vi "SelectPatternDialog.vi"(0 "GraphIn":refnum<class "Graph.lvclass">, 1 "SelectedNodes":refnum<class "AbstractNode.lvclass">[](array[class]), 5 "error in":errorcluster) -> (14 "GraphOut":refnum<class "Graph.lvclass">, 15 "Cancelled":bool, 16 "NodesOut":T3[](array[typedef]), 17 "LinksOut":T1[](array[typedef]), 18 "NodeIndexies":i32[](array[numeric]), 19 "error out":errorcluster)   [LabVIEW 2020]
uses:
  <resource>/Framework/Providers/Open_GDS/UML/Graph_class/Graph.lvclass
  <resource>/Framework/Providers/Open_GDS/UML/AbstractNode_class/AbstractNode.lvclass
  <resource>/Framework/Providers/Open_GDS/UML/DesignPattern/SubVIs/DesignPatterns_Node.ctl
  <resource>/Framework/Providers/Open_GDS/UML/DesignPattern/SubVIs/DesignPatterns_NodeType.ctl
  <resource>/Framework/Providers/Open_GDS/UML/DesignPattern/SubVIs/DesignPatterns_Link.ctl
  <resource>/Framework/Providers/Open_GDS/UML/DesignPattern/SubVIs/DesignPatterns_LinkType.ctl
  <resource>/Framework/Providers/Open_GDS/UML/Graphics_class/Graphics.lvclass
  <resource>/Framework/Providers/Open_GDS/UML/Grid_class/Grid.lvclass
  <resource>/Framework/Providers/Open_GDS/UML/ClassDiagramGraph_class/ClassDiagramGraph.lvclass
  C:/Program Files (x86)/National Instruments/LabVIEW 2020/resource/Framework/Providers/Open_GDS/UML/Graph_class/Graph.lvclass
  <resource>/Framework/Providers/Open_GDS/UML/DesignPattern/SubVIs/DesignPatterns_Pattern.ctl
  <resource>/Framework/Providers/Open_GDS/UML/Graphics_class/LvFontType.ctl
  <resource>/Framework/Providers/Open_GDS/UML/Graphics_class/FontType.ctl
  <resource>/Framework/Providers/Open_GDS/UML/ClassNode_class/ClassNode.lvclass
  <resource>/Framework/Providers/Open_GDS/UML/DesignPattern/SubVIs/DesignPatterns_ClassNodeData.ctl
  <resource>/Framework/Providers/Open_GDS/UML/DesignPattern/SubVIs/DesignPatterns_Attribute.ctl
  <resource>/Framework/Providers/Open_GDS/UML/DesignPattern/SubVIs/DesignPatterns_Method.ctl
  <vilib>/Platform/browser.llb/Open URL in Default Browser (string).vi
panel:
  in  "OpenPatternFile":bool
  in  "Refresh":bool
  in  "Ring 10":u16(ring) items=["<Select>"]
  in  "Ring 9":u16(ring) items=["<Select>"]
  in  "Ring 8":u16(ring) items=["<Select>"]
  in  "Ring 7":u16(ring) items=["<Select>"]
  in  "Help":bool
  in  "Cancel":bool
  in  "OK":bool
  out "Nodes":cluster{"Name":string, "Desc":string}[](array[cluster])
  out "Pattern description":string
  out "NewVal":string
  in  "Design Patterns":string(tree)
  in  "InterfaceNames":string[](array[string])
  in  "PackageNames":string[](array[string])
  out "ClassNames":string[](array[string])
  in  "Ring 6":u16(ring) items=["<Select>"]
  in  "Ring 5":u16(ring) items=["<Select>"]
  in  "Ring 4":u16(ring) items=["<Select>"]
  in  "Ring 3":u16(ring) items=["<Select>"]
  in  "Ring 2":u16(ring) items=["<Select>"]
  in  "Ring 1":u16(ring) items=["<Select>"]
  out "Picture":picture
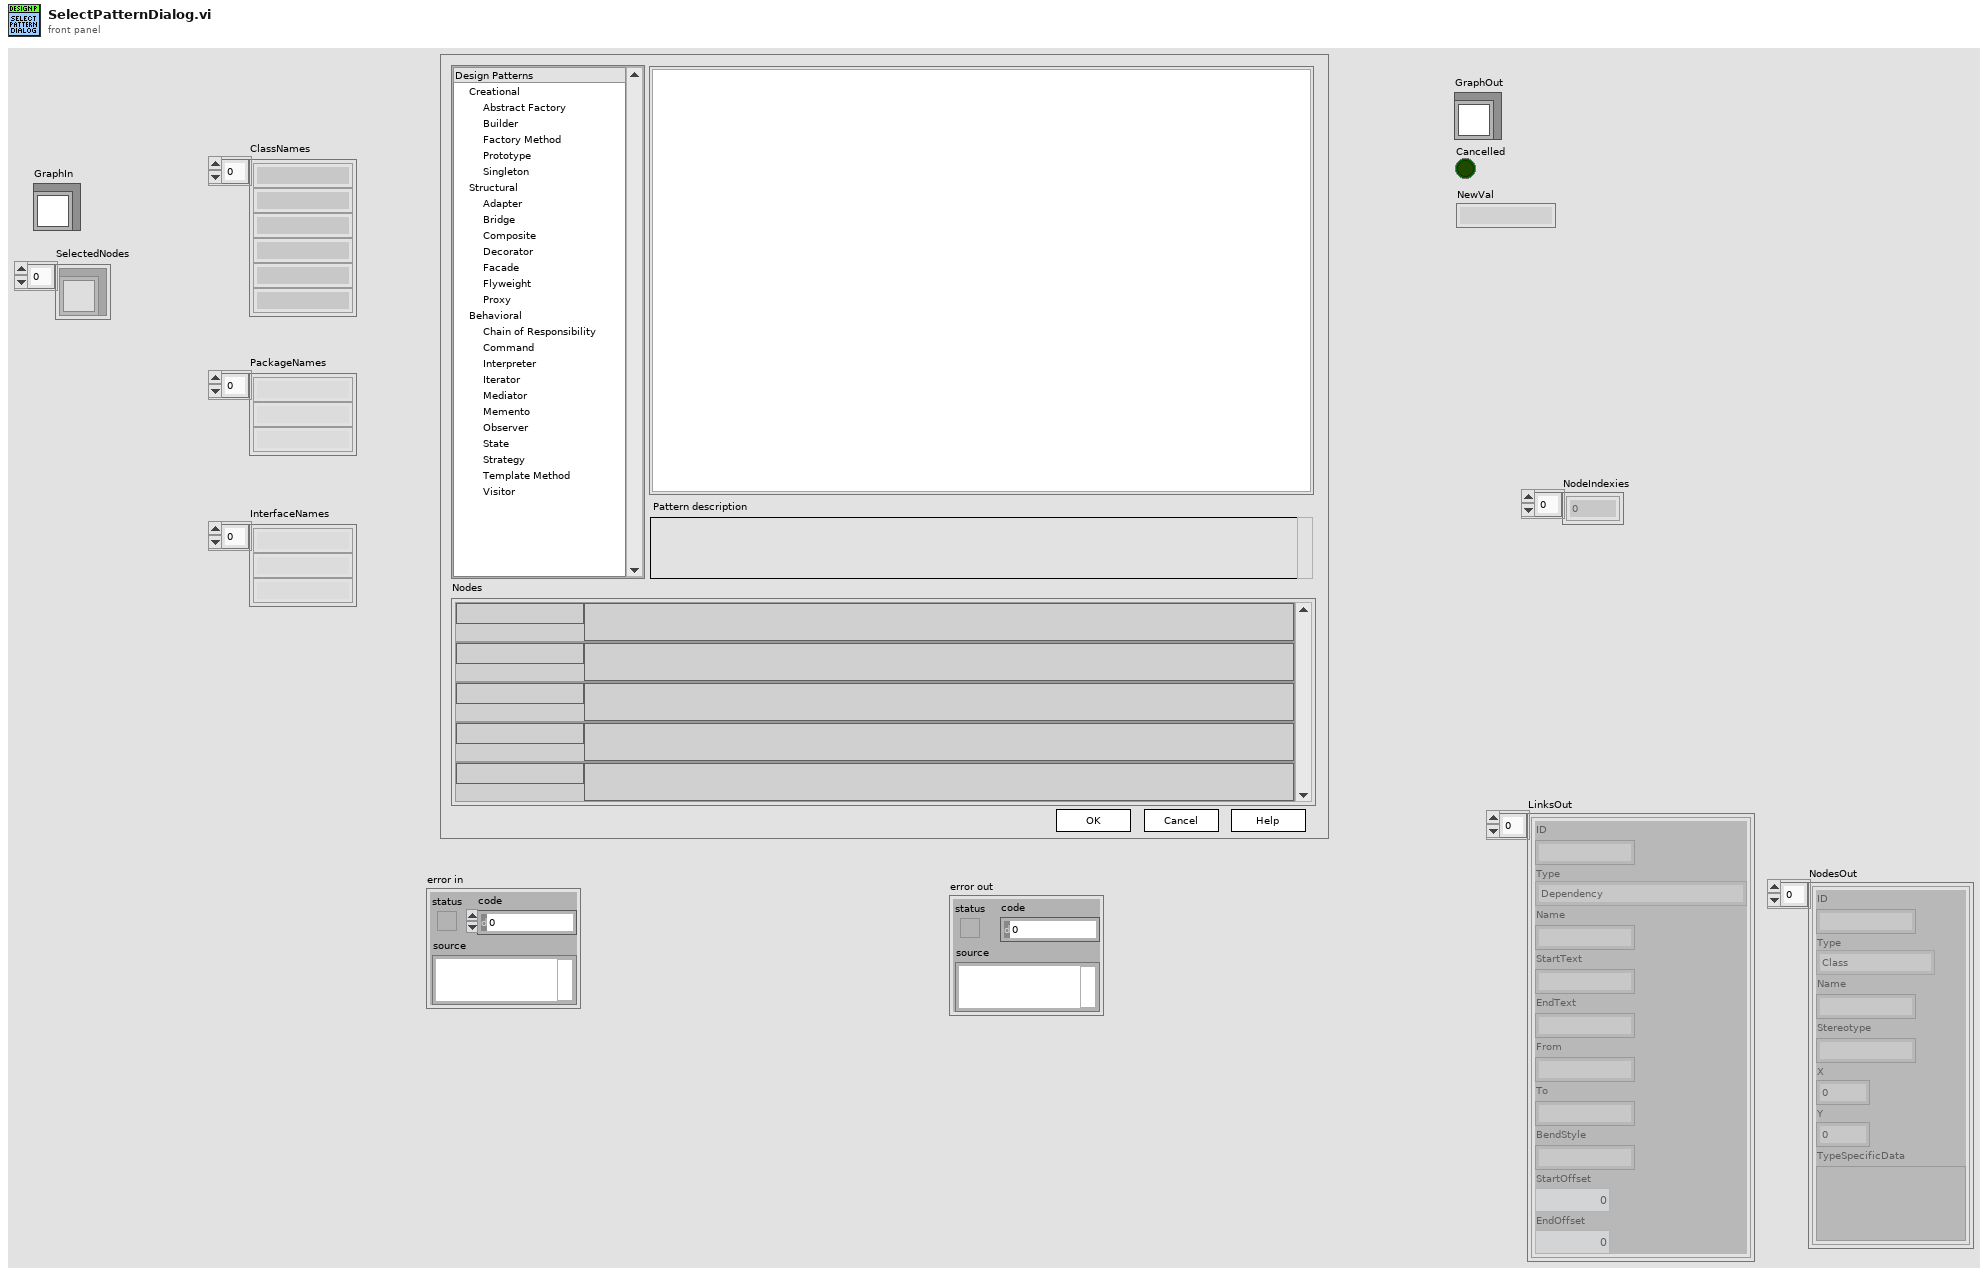
[diagram p1: front panel]
types:
  T1 = typedef "DesignPatterns_Link.ctl" = cluster{"ID":string, "Type":T2, "Name":string, "StartText":string, "EndText":string, "From":string, "To":string, "BendStyle":string, "StartOffset":i32, "EndOffset":i32}
  T2 = typedef "DesignPatterns_LinkType.ctl" = enum16{"Dependency", "Inheritance", "Interface", "Association", "Aggregation", "CompositeAggregation"}
  T3 = typedef "DesignPatterns_Node.ctl" = cluster{"ID":string, "Type":T4, "Name":string, "Stereotype":string, "X":i32, "Y":i32, "TypeSpecificData":variant}
  T4 = typedef "DesignPatterns_NodeType.ctl" = enum16{"Class", "Interface", "Note", "Package"}
  T5 = typedef "DesignPatterns_Pattern.ctl" = cluster{"Version":string, "ID":string, "Name":string, "Category":string, "Help":string, "Desc":string}
  T6 = cluster{"Cancelled":bool, "Event":refnum<event-registration>, "CtrlRefs":refnum<vi>[], "PIDs":string[], "Graphics":refnum<class "Graphics.lvclass">, "Grid":refnum<class "Grid.lvclass">, "Diagram":refnum<class "ClassDiagramGraph.lvclass">, "ClassNodes":T3[], "ClassSelected":bool[], "NodeIndexies":i32[], "Patterns":cluster{"PatternFile":path, "Pattern":T5, "Nodes":T3[], "Links":T1[], "stripped path":path, "HelpExist":bool}[], "Interface?":bool[]}
  T7 = typedef "Graphics.lvclass/FontType.ctl" = cluster{"Font Name:":string, "Size":i16, "Strikeout?":bool, "Italic?":bool, "Underline?":bool, "Outline?":bool, "Shadow?":bool, "Bold?":bool}
  T8 = typedef "Graphics.lvclass/LvFontType.ctl" = enum16{"User-specified Font", "Application Font", "System Font", "Dialog Font"}
  T9 = cluster{path, "Pattern":T5, "Nodes":T3[], "Links":T1[], "stripped path":path, "file or folder exists?":bool}[]
  T10 = typedef "DesignPatterns_ClassNodeData.ctl" = cluster{"Description":string, "Attributes":T11[], "Methods":T12[]}
  T11 = typedef "DesignPatterns_Attribute.ctl" = cluster{"ID":string, "Name":string}
  T12 = typedef "DesignPatterns_Method.ctl" = cluster{"ID":string, "Name":string}
  T13 = typedef "Rectangle Rectangle2D.ctl" = cluster{"x":dbl, "y":dbl, "width":dbl, "height":dbl}
  T14 = cluster{path, "Pattern":T5, "Nodes":T3[], "Links":T1[], "stripped path":path, "file or folder exists?":bool}
  T15 = cluster{"PatternFile":path, "Pattern":T5, "Nodes":T3[], "Links":T1[], "stripped path":path, "HelpExist":bool}[]
  T16 = cluster{"PatternFile":path, "Pattern":T5, "Nodes":T3[], "Links":T1[], "stripped path":path, "HelpExist":bool}
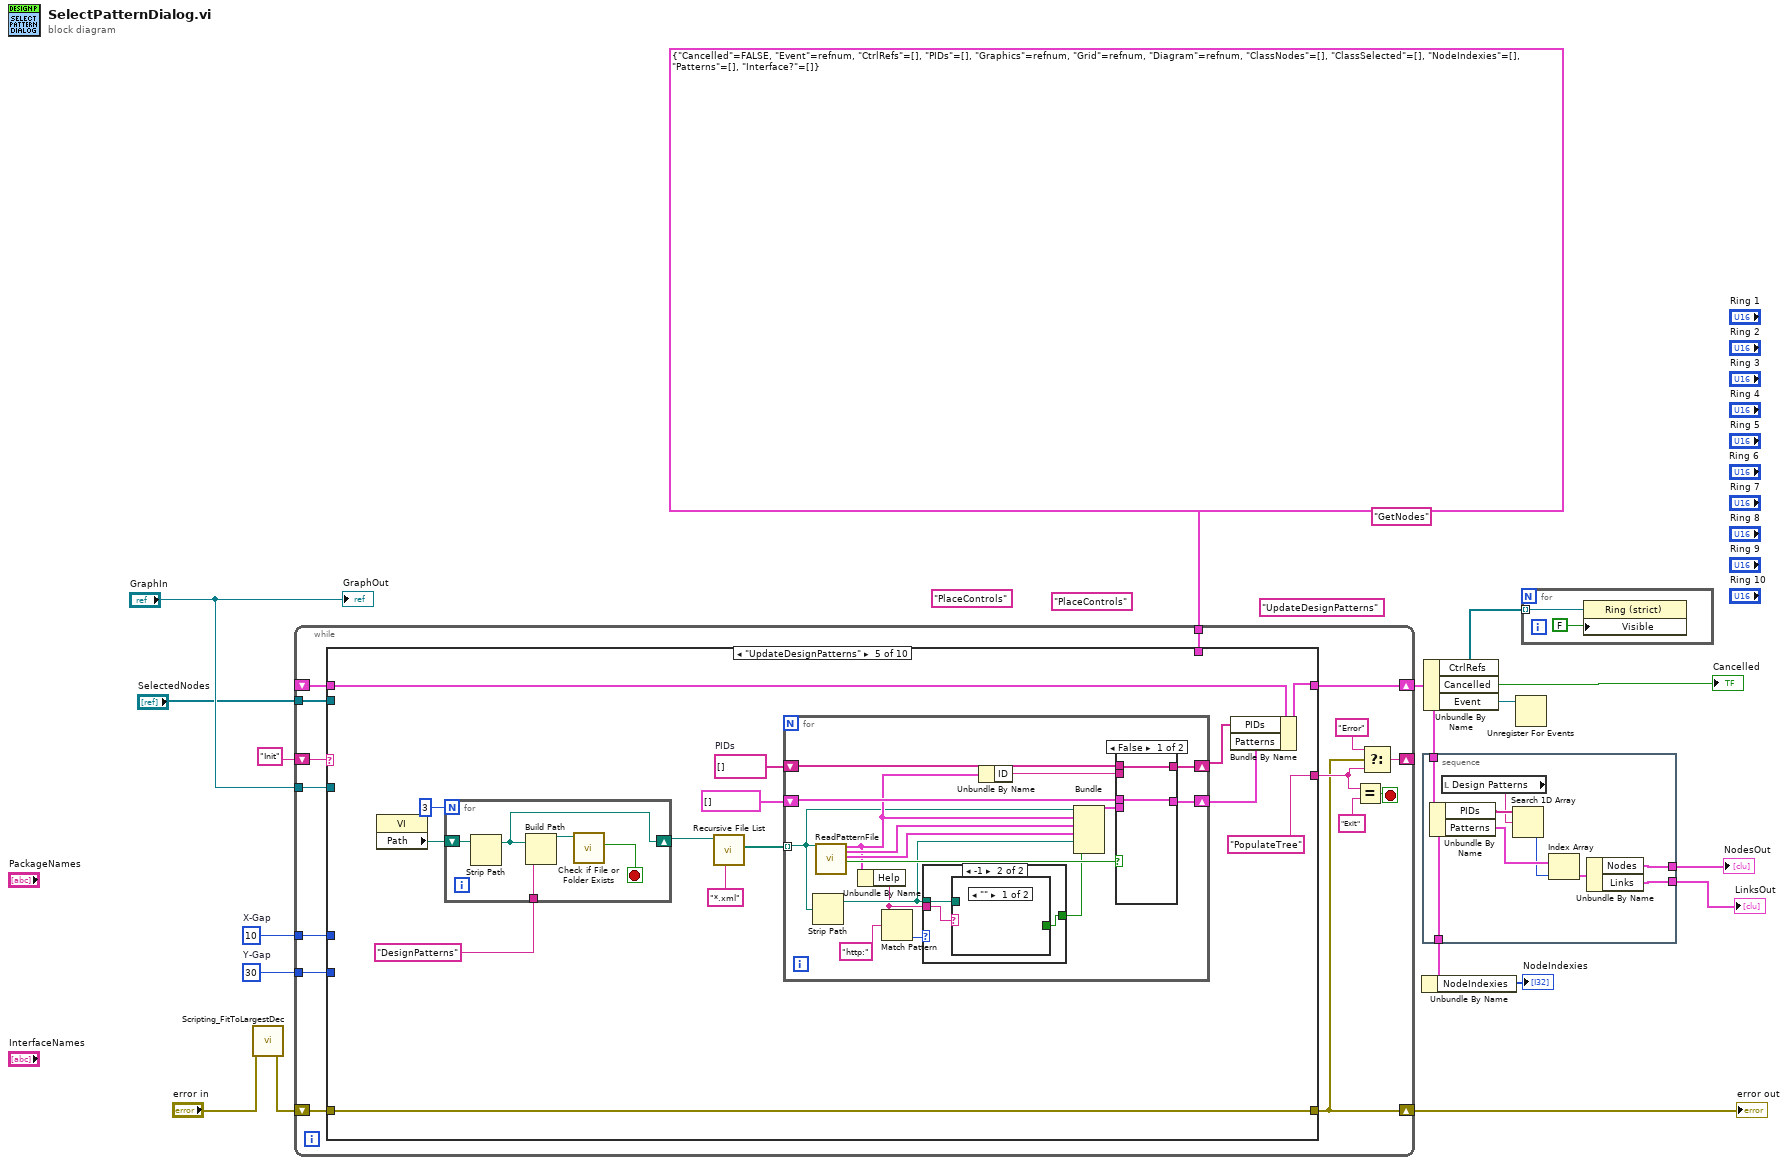
[diagram p0: block diagram]
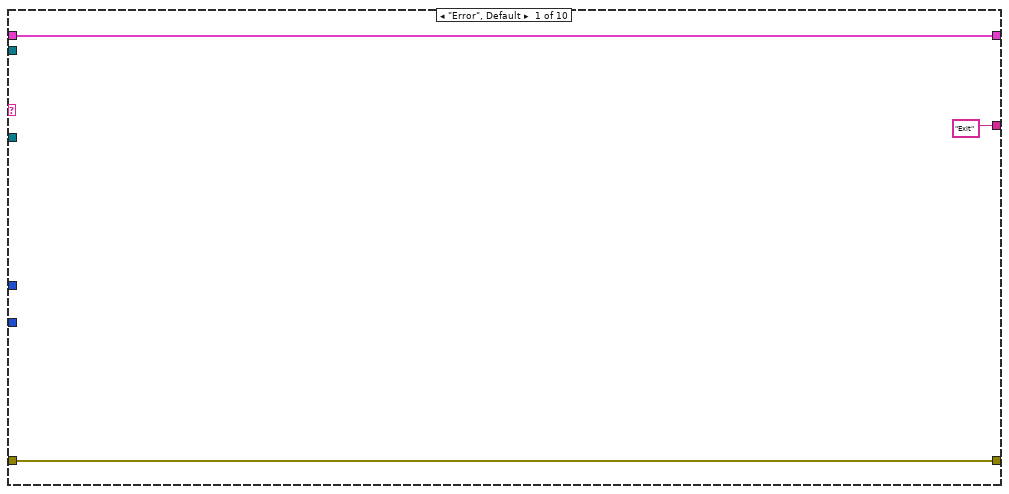
[diagram p2: hidden frame]
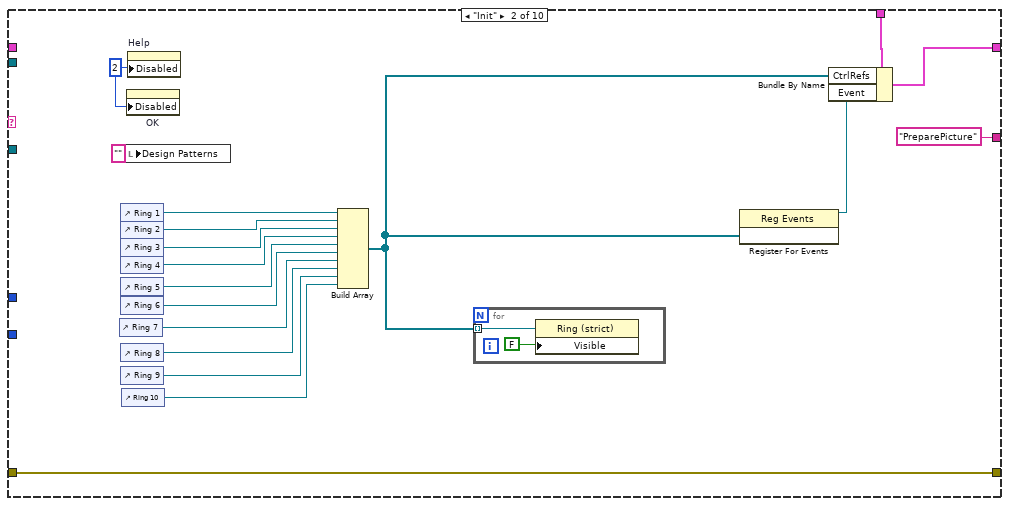
[diagram p3: hidden frame]
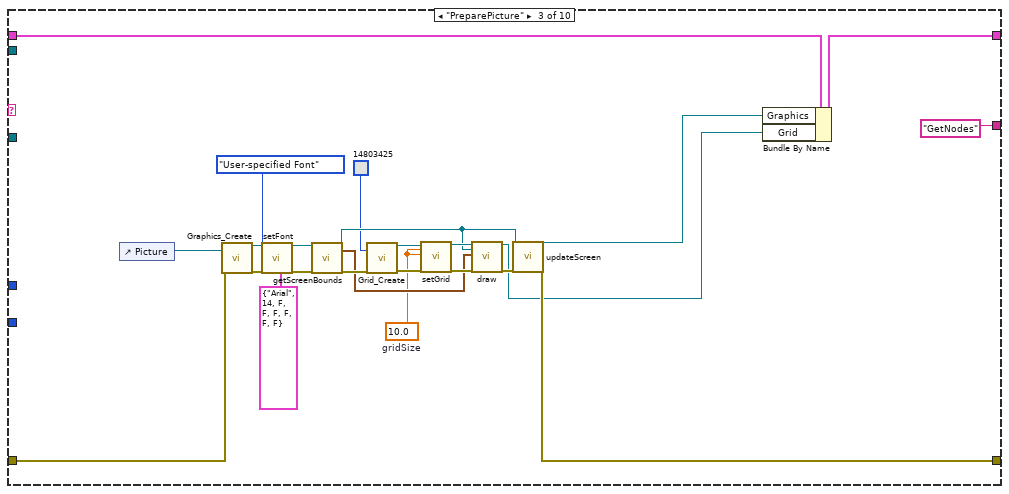
[diagram p4: hidden frame]
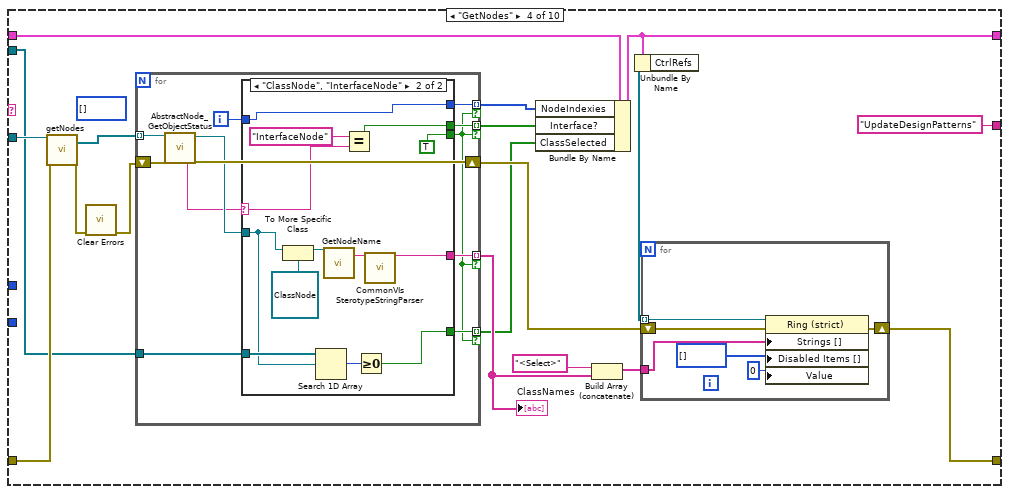
[diagram p5: hidden frame]
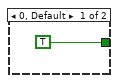
[diagram p7: hidden frame]
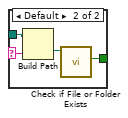
[diagram p8: hidden frame]
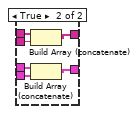
[diagram p9: hidden frame]
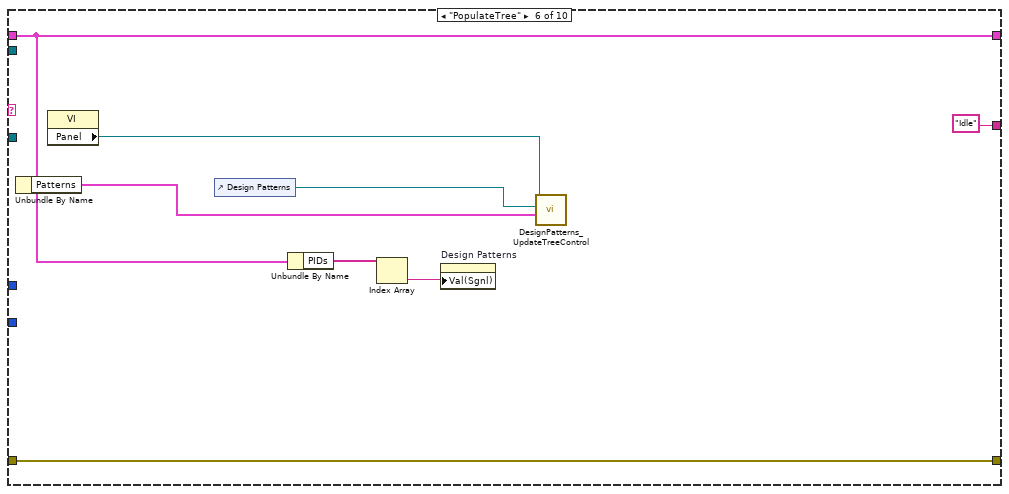
[diagram p10: hidden frame]
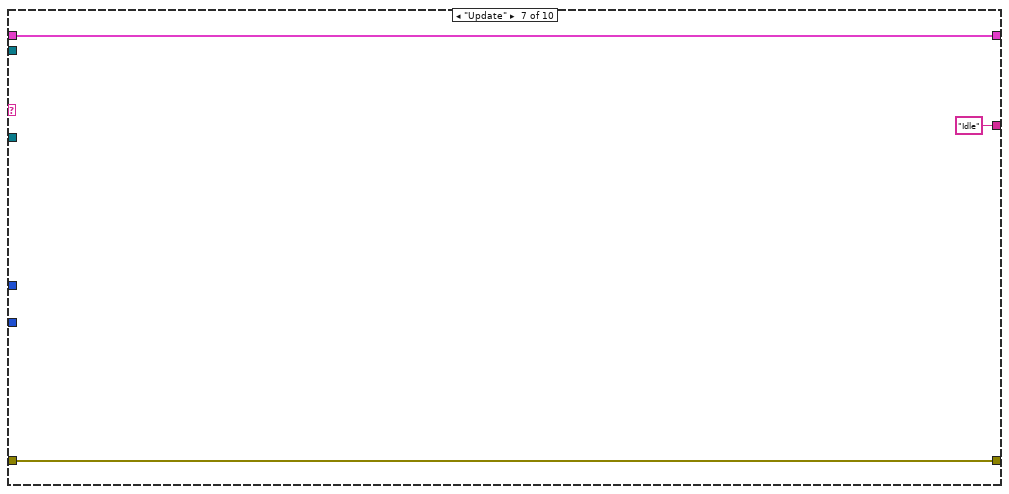
[diagram p11: hidden frame]
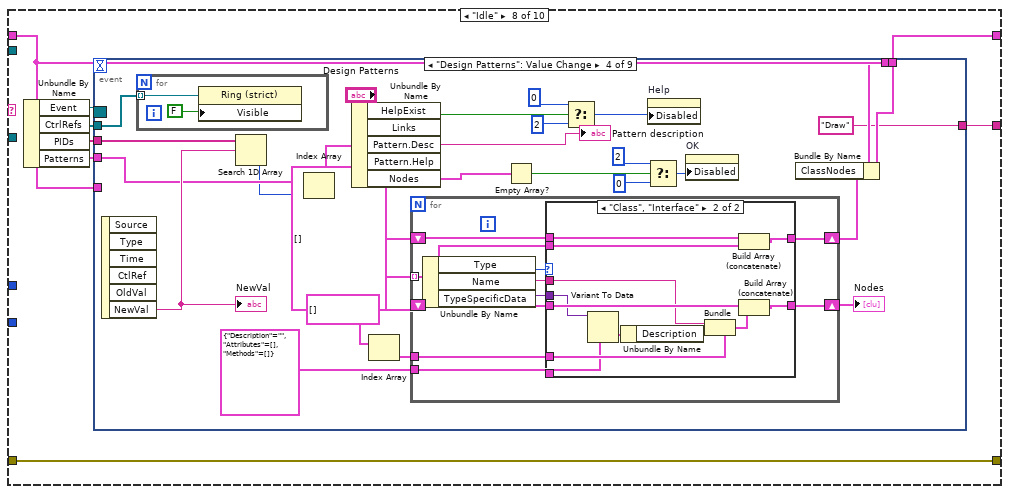
[diagram p12: hidden frame]
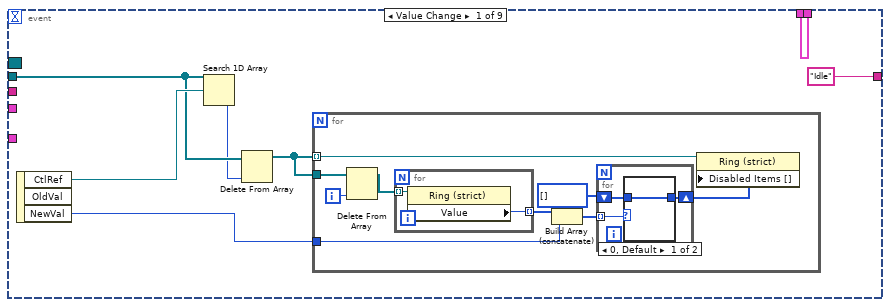
[diagram p13: hidden frame]
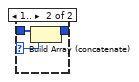
[diagram p14: hidden frame]
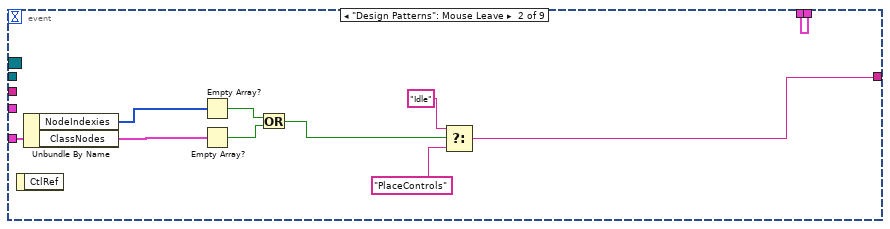
[diagram p15: hidden frame]
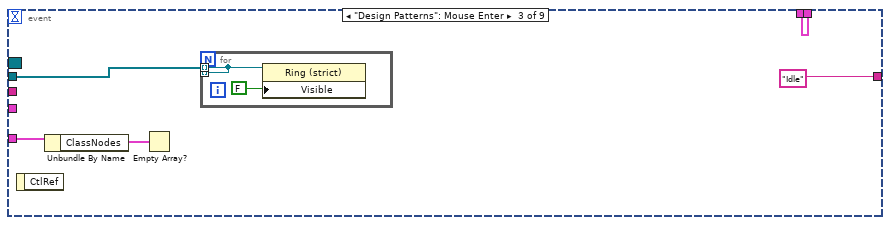
[diagram p16: hidden frame]
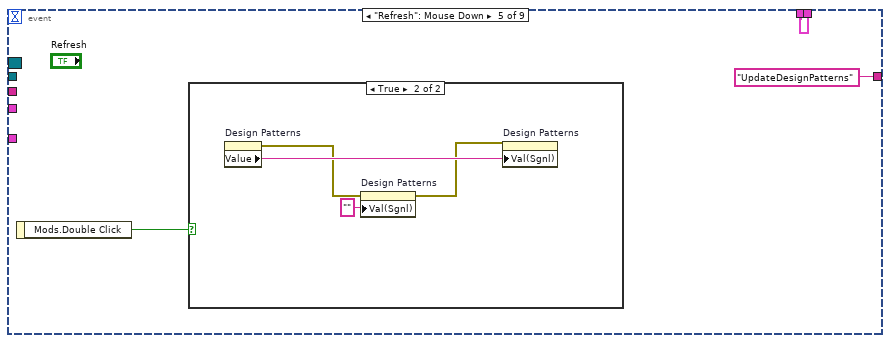
[diagram p18: hidden frame]
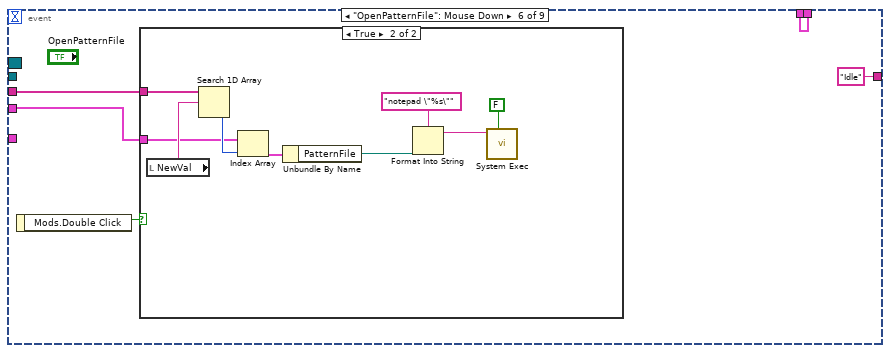
[diagram p20: hidden frame]
diagram:
  (unwired) "PlaceControls"
  w8 = 30  # Y-Gap
  w9 = 10  # X-Gap
  (unwired) "GetNodes"
  (unwired) "UpdateDesignPatterns"
  (unwired) "PlaceControls"
  n1 = call <resource>:"Scripting_FitToLargestDec.vi"("error in (no error)"="error in") -> ("error out"=w10:errorcluster)  [unwired: 5 in, 1 out]
  n2 = while {
    shift-right: [w25] -> w16
    shift-left: w10 -> [w32]
    shift-right: [w30] -> _
    shift-left: "Init" -> [w31]
    shift-right: [w24] -> w6
    shift-left: _ -> [w23]
    tunnel: T6 {"Cancelled"=FALSE, "Event"=refnum, "CtrlRefs"=[], "PIDs"=[], "Graphics"=refnum, "Grid"=refnum, "Diagram"=refnum, "ClassNodes"=[], "ClassSelected"=[], "NodeIndexies"=[], "Patterns"=[], "Interface?"=[]} -> [w22]
    tunnel: "GraphIn" -> [w21]
    tunnel: w9 -> [w20]
    tunnel: w8 -> [w19]
    tunnel: "SelectedNodes" -> [w18]
    stop <- w29 stop-if-true
    n3 = case shown="\"UpdateDesignPatterns\"" w31 {
      tunnel: w32 -> [w35 w52 w63 w91 w132 w185 w188 w196 w365 w405]
      tunnel: [w35 w52 w62 w90 w132 w185 w188 w196 w367 w401] -> w25
      tunnel: ["Exit" "PreparePicture" "GetNodes" "UpdateDesignPatterns" "PopulateTree" "Idle" "Idle" w197 "Idle" "Idle"] -> w26
      tunnel: [w33 w51 w56 w86 w134 w182 w189 w198 w387 w399] -> w24
      tunnel: w23 -> [w33 _ w57 w87 w136 w182 w189 w191 w387 w399]
      tunnel: w22 -> [_ w43 _ _ _ _ _ _ _ _]
      tunnel: w21 -> [_ _ _ w93 _ _ _ _ _ _]
      tunnel: w20 -> [_ _ _ _ _ _ _ _ w360 w412]
      tunnel: w19 -> [_ _ _ _ _ _ _ _ w359 w411]
      tunnel: w18 -> [_ _ _ w88 _ _ _ _ _ w404]
      frame "Error", Default {
      }
      frame "Init" {
        w42 = u8 2 ("Disabled")
        n4 = control-ref of="Ring 7"() -> (w39:refnum<vi>)
        n5 = control-ref of="Ring 1"() -> (w45:refnum<vi>)
        n6 = control-ref of="Ring 2"() -> (w46:refnum<vi>)
        n7 = control-ref of="Ring 3"() -> (w47:refnum<vi>)
        n8 = control-ref of="Ring 4"() -> (w48:refnum<vi>)
        n9 = control-ref of="Ring 5"() -> (w49:refnum<vi>)
        n10 = control-ref of="Ring 6"() -> (w50:refnum<vi>)
        n11 = control-ref of="Ring 8"() -> (w38:refnum<vi>)
        n12 = control-ref of="Ring 9"() -> (w37:refnum<vi>)
        n13 = control-ref of="Ring 10"() -> (w36:refnum<vi>)
        n14 = local write "Design Patterns"("" ("Design Patterns")) -> ()
        n15 = property on="OK" class="Bool"("Disabled"=w42) -> ()  [unwired: 2 in, 2 out]
        n16 = property on="Help" class="Bool"("Disabled"=w42) -> ()  [unwired: 2 in, 2 out]
        n17 = Build Array(w45, w46, w47, w48, w49, w50, w39, w38, w37, w36) -> (w40:refnum<vi>[])
        n18 = for {
          tunnel: w40 -> [w55] mode=indexing
          n19 = property class="Ring (strict)"(reference=w55, "Visible"=FALSE) -> ()  [unwired: 1 in, 2 out]
        }
        n20 = register-events(w40) -> (reference out=w44:refnum<event-registration>)  [unwired: 2 in, 1 out]
        n21 = Bundle By Name(cluster=w43, "CtrlRefs"=w40, "Event"=w44) -> (w51:T6)
      }
      frame "PreparePicture" {
        w64 = 10.0  # gridSize
        n22 = control-ref of="Picture"() -> (w60:refnum<vi>)
        n23 = call <resource>:"Graphics_Create.vi"("screenRef"=w60, "error in (no error)"=w63) -> ("reference out"=w73:refnum<class "Graphics.lvclass">, "error out"=w72:errorcluster)  [unwired: 1 in, 15 out]
        n24 = call <resource>:"setFont.vi"("reference"=w73, "fontType"=LvFontType."User-specified Font", "font"=T7 {"Font Name:"="Arial", "Size"=14, "Strikeout?"=FALSE, "Italic?"=FALSE, "Underline?"=FALSE, "Outline?"=FALSE, "Shadow?"=FALSE, "Bold?"=FALSE}, "error in (no error)"=w72) -> ("reference out"=w71:refnum<class "Graphics.lvclass">, "error out"=w70:errorcluster)  [unwired: 14 out]
        n25 = call <resource>:"getScreenBounds.vi"("reference"=w71, "error in (no error)"=w70) -> ("reference out"=w74:refnum<class "Graphics.lvclass">, "bounds"=w67:T13, "error out"=w79:errorcluster)  [unwired: 15 out]
        n26 = call <resource>:"Grid_Create.vi"("gridColor"=u32 14803425, "error in (no error)"=w79) -> ("reference out"=w76:refnum<class "Grid.lvclass">, "error out"=w77:errorcluster)  [unwired: 1 in, 15 out]
        n27 = call <resource>:"setGrid.vi"("reference"=w76, "gridX"=w64, "gridY"=w64, "error in (no error)"=w77) -> ("reference out"=w75:refnum<class "Grid.lvclass">, "error out"=w78:errorcluster)  [unwired: 14 out]
        n28 = call-dynamic "draw.vi"("reference"=w75, "graphics"=w74, "bounds"=w67, "error in (no error)"=w78) -> ("reference out"=w58:refnum<class "Grid.lvclass">, "error out"=w66:errorcluster)  [unwired: 14 in]
        n29 = call <resource>:"updateScreen.vi"("reference"=w74, "error in (no error)"=w66) -> ("reference out"=w59:refnum<class "Graphics.lvclass">, "error out"=w62:errorcluster)  [unwired: 16 out]
        n30 = Bundle By Name(cluster=w57, "Graphics"=w59, "Grid"=w58) -> (w56:T6)
      }
      frame "GetNodes" {
        (unwired) i32[] []
        n31 = call-dynamic "getNodes.vi"("reference"=w93, "error in (no error)"=w91) -> ("nodes"=w92:refnum<class "AbstractNode.lvclass">[], "error out"=w81:errorcluster)  [unwired: 15 in, 1 out]
        n32 = call <vilib>:"Clear Errors.vi"("error in (no error)"=w81) -> ("error out"=w80:errorcluster)  [unwired: 5 in, 1 out]
        n33 = for {
          shift-right: [w107] -> w89
          shift-left: w80 -> [w109]
          tunnel: w92 -> [w108] mode=indexing
          tunnel: w88 -> [w105]
          tunnel: [w102] -> w85 mode=indexing if=w98
          tunnel: [w101] -> w84 mode=indexing if=w98
          tunnel: [w100] -> w83 mode=indexing if=w98
          tunnel: [w99] -> w82 mode=indexing if=w98
          i -> [w104]
          n34 = call <resource>:"AbstractNode_GetObjectStatus.vi"("reference in"=w108, "error in (no error)"=w109) -> ("Class name"=w103:string, "reference out"=w106:refnum<class "AbstractNode.lvclass">, "error out"=w107:errorcluster)  [unwired: 15 out]
          n35 = case shown="\"ClassNode\", \"InterfaceNode\"" w103 {
            selector: w103 -> [_ w116]
            tunnel: w106 -> [_ w118]
            tunnel: w105 -> [_ w119]
            tunnel: [_ w112] -> w101
            tunnel: w104 -> [_ w112]
            tunnel: [_ w114] -> w102
            tunnel: [_ TRUE] -> w98
            tunnel: [_ w111] -> w100
            tunnel: [_ w110] -> w99
            frame Default {
            }
            frame "ClassNode", "InterfaceNode" {
              n36 = To More Specific Class(target class=refnum<class "ClassNode.lvclass"> refnum ("reference"), reference=w118) -> (specific class reference=w121:refnum<class "ClassNode.lvclass">)  [unwired: 1 in, 1 out]
              n37 = Search 1D Array(1D array=w119, element=w118) -> (index of element=w117:i32)  [unwired: 1 in]
              n38 = call-dynamic "GetNodeName.vi"("reference in"=w121) -> ("String"=w120:string)  [unwired: 16 in, 2 out]
              n39 = Equal?(x="InterfaceNode", y=w116) -> (x = y?=w114:bool)
              n40 = Greater Or Equal To 0?(x=w117) -> (x >= 0?=w110:bool)
              n41 = call <resource>:"CommonVIs SterotypeStringParser.vi"("SterotypeStringIn"=w120) -> ("Name"=w111:string)  [unwired: 18 out]
            }
          }
        }
        "ClassNames" <- w83
        n42 = Bundle By Name(cluster=w87, "NodeIndexies"=w84, "Interface?"=w85, "ClassSelected"=w82) -> (w86:T6)
        n43 = Build Array (concatenate)("<Select>", w83) -> (w96:string[])
        n44 = Unbundle By Name(w86) -> ("CtrlRefs"=w95:refnum<vi>[])
        n45 = for {
          tunnel: w95 -> [w128] mode=indexing
          tunnel: w96 -> [w127]
          shift-right: [w123] -> w90
          shift-left: w89 -> [w124]
          n46 = property class="Ring (strict)"(reference=w128, error in=w124, "Strings []"=w127, "Disabled Items []"=i32[] [], "Value"=u16 0) -> (error out=w123:errorcluster)  [unwired: 1 out]
        }
      }
      frame "UpdateDesignPatterns" {
        w131 = string[] []  # PIDs
        n47 = property class="VI"() -> ("Path"=w140:path)  [unwired: 2 in, 2 out]
        n48 = for {
          N: 3 -> [_]
          tunnel: "DesignPatterns" ("name or relative path") -> [w179]
          shift-right: [w175] -> w139
          shift-left: w140 -> [w176]
          stop <- w177 stop-if-true
          n49 = Strip Path(path=w176) -> (stripped path=w175:path)  [unwired: 1 out]
          n50 = Build Path(base path=w175, name or relative path=w179) -> (appended path=w178:path)
          n51 = call <vilib>:"Check if File or Folder Exists.vi"("path"=w178) -> ("file or folder exists?"=w177:bool)  [unwired: 1 in, 9 out]
        }
        n52 = call <vilib>:"Recursive File List.vi"("pattern"="*.xml", "Folder Path"=w139) -> ("All Files in Dir"=w137:path[])  [unwired: 2 in, 7 out]
        n53 = for {
          tunnel: w137 -> [w143] mode=indexing
          shift-right: [w154] -> w135
          shift-left: T9 [] -> [w156]
          shift-right: [w151] -> w130
          shift-left: w131 -> [w150]
          n54 = Strip Path(path=w143) -> (stripped path=w145:path)  [unwired: 1 out]
          n55 = call <resource>:"ReadPatternFile.vi"("PatternsXMLFileIn"=w143) -> ("Pattern"=w149:T5, "Nodes"=w158:T3[], "Links"=w157:T1[], "Valid"=w153:bool)  [unwired: 2 in, 13 out]
          n56 = Unbundle By Name(w149) -> ("Help"=w144:string)
          n57 = Match Pattern(string=w144, regular expression="http:") -> (offset past match=w147:i32)  [unwired: 4 out]
          n58 = case shown="-1" w147 {
            tunnel: [TRUE w160] -> w146
            tunnel: w145 -> [_ w162]
            tunnel: w144 -> [_ w161]
            frame 0, Default {
            }
            frame -1 {
              n59 = case shown="\"\"" w161 {
                selector: w161 -> [_ w164]
                tunnel: w162 -> [_ w165]
                tunnel: [_ w163] -> w160
                frame "" {
                }
                frame Default {
                  n60 = Build Path(base path=w165, name or relative path=w164) -> (appended path=w166:path)
                  n61 = call <vilib>:"Check if File or Folder Exists.vi"("path"=w166) -> ("file or folder exists?"=w163:bool)  [unwired: 1 in, 9 out]
                }
              }
            }
          }
          n62 = Unbundle By Name(w149) -> ("ID"=w152:string)
          n63 = Bundle(w143, "Pattern"=w149, "Nodes"=w158, "Links"=w157, "stripped path"=w145, "file or folder exists?"=w146) -> (w155:T14)  [unwired: 1 out]
          n64 = case shown="False" w153 {
            tunnel: w156 -> [w168 w174]
            tunnel: w155 -> [_ w173]
            tunnel: [w168 w172] -> w154
            tunnel: w152 -> [_ w171]
            tunnel: [w167 w170] -> w151
            tunnel: w150 -> [w167 w169]
            frame False {
            }
            frame True {
              n65 = Build Array (concatenate)(w169, w171) -> (w170:string[])
              n66 = Build Array (concatenate)(w174, w173) -> (w172:T9)
            }
          }
        }
        n67 = Bundle By Name(cluster=w136, "PIDs"=w130, "Patterns"=w135) -> (w134:T6)
      }
      frame "PopulateTree" {
        n68 = Unbundle By Name(w182) -> ("Patterns"=w184:T15)
        n69 = property class="VI"() -> ("Panel"=w187:refnum<vi>)  [unwired: 2 in, 2 out]
        n70 = control-ref of="Design Patterns"() -> (w183:refnum<vi>)
        n71 = Unbundle By Name(w182) -> ("PIDs"=w181:string[])
        n72 = Index Array(array=w181) -> (element=w180:string)  [unwired: 1 in]
        n73 = property on="Design Patterns" class="Tree (strict)"("Val(Sgnl)"=w180) -> ()  [unwired: 2 in, 2 out]
        n74 = call <resource>:"DesignPatterns_UpdateTreeControl.vi"("Patterns"=w184, "Tree Refnum"=w183, "Panel"=w187) -> ()  [unwired: 9 out]
      }
      frame "Update" {
      }
      frame "Idle" {
        n75 = Unbundle By Name(w191) -> ("Event"=w195:refnum<event-registration>, "CtrlRefs"=w194:refnum<vi>[], "PIDs"=w193:string[], "Patterns"=w192:T15)
        n76 = event shown="[3] \"Design Patterns\": Value Change" {
          selector: w195 -> [_ _ _ _ _ _ _ _ _]
          dyn-events: _ -> [_ _ _ _ _ _ _ _ _]
          timeout: _ -> [_ _ _ _ _ _ _ _ _]
          tunnel: w191 -> [w200 w233 w236 w246 w293 w300 w315 w332 w342]
          tunnel: [w200 w233 w236 w245 w293 w300 w315 w331 w341] -> w198
          tunnel: ["Idle" w228 "Idle" ("t") "Draw" "UpdateDesignPatterns" "Idle" ("t") "Idle" "Exit" "Exit"] -> w197
          tunnel: w194 -> [w204 _ w234 w247 _ _ _ _ _]
          tunnel: w193 -> [_ _ _ w265 _ w302 w322 _ _]
          tunnel: w192 -> [_ _ _ w263 _ w301 w320 _ _]
          tunnel: w191 -> [_ w232 w237 _ _ _ _ _ w338]
          event Value Change {
            n77 = event-data() -> ("CtlRef"=w205:refnum<vi>, "NewVal"=w201:u16)  [unwired: 2 out]
            n78 = Search 1D Array(1D array=w204, element=w205) -> (index of element=w203:i32)  [unwired: 1 out]
            n79 = Delete From Array(array=w204, index=w203) -> (array with subset deleted=w202:refnum<vi>[])  [unwired: 1 in, 1 out]
            n80 = for {
              tunnel: w202 -> [w214] mode=indexing
              tunnel: w202 -> [w213]
              tunnel: w201 -> [w209]
              i -> [w212]
              n81 = Delete From Array(array=w213, index=w212) -> (array with subset deleted=w211:refnum<vi>[])  [unwired: 1 in, 1 out]
              n82 = for {
                tunnel: w211 -> [w223] mode=indexing
                tunnel: [w222] -> w210 mode=indexing
                n83 = property class="Ring (strict)"(reference=w223) -> ("Value"=w222:u16)  [unwired: 1 in, 2 out]
              }
              n84 = Build Array (concatenate)(w210, w209) -> (w208:u16[])
              n85 = for {
                tunnel: w208 -> [w217] mode=indexing
                shift-right: [w215] -> w206
                shift-left: u16[] [] -> [w216]
                n86 = case shown="0, Default" w217 {
                  selector: w217 -> [_ w219]
                  tunnel: w216 -> [w218 w221]
                  tunnel: [w218 w220] -> w215
                  frame 0, Default {
                  }
                  frame 1.. {
                    n87 = Build Array (concatenate)(w221, w219) -> (w220:u16[])
                  }
                }
              }
              n88 = property class="Ring (strict)"(reference=w214, "Disabled Items []"=w206) -> ()  [unwired: 1 in, 2 out]
            }
          }
          event "Design Patterns": Mouse Leave {
            n89 = event-data() -> ()  [unwired: 2 out]
            n90 = Unbundle By Name(w232) -> ("NodeIndexies"=w227:i32[], "ClassNodes"=w231:T3[])
            n91 = Empty Array?(array=w227) -> (empty?=w226:bool)
            n92 = Empty Array?(array=w231) -> (empty?=w225:bool)
            n93 = Or(x=w226, y=w225) -> (x .or. y?=w224:bool)
            n94 = Select(t="Idle", s=w224, f="PlaceControls") -> (s? t:f=w228:string)
          }
          event "Design Patterns": Mouse Enter {
            n95 = event-data() -> ()  [unwired: 2 out]
            n96 = Unbundle By Name(w237) -> ("ClassNodes"=w238:T3[])
            n97 = Empty Array?(array=w238) -> ()  [unwired: 1 out]
            n98 = for {
              tunnel: [w239] -> _ mode=indexing
              tunnel: w234 -> [w239] mode=indexing
              n99 = property class="Ring (strict)"(reference=w239, "Visible"=FALSE) -> ()  [unwired: 1 in, 2 out]
            }
          }
          event "Design Patterns": Value Change {
            w260 = cluster{"Name":string, "Desc":string}[] [] ("Nodes")
            n100 = event-data() -> ("NewVal"=w264:string)  [unwired: 6 out]
            "NewVal" <- w264
            n101 = for {
              tunnel: w247 -> [w267] mode=indexing
              n102 = property class="Ring (strict)"(reference=w267, "Visible"=FALSE) -> ()  [unwired: 1 in, 2 out]
            }
            n103 = Search 1D Array(1D array=w265, element=w264) -> (index of element=w262:i32)  [unwired: 1 out]
            n104 = Index Array(array=w263, index=w262) -> (element=w261:T16)
            n105 = Unbundle By Name(w261) -> ("HelpExist"=w256:bool, "Pattern.Desc"=→"Pattern description":string, "Nodes"=w250:T3[])  [unwired: 2 out]
            n106 = Index Array(array=w260) -> (element=w259:cluster{"Name":string, "Desc":string})  [unwired: 1 in]
            n107 = for {
              tunnel: w250 -> [w269] mode=indexing
              shift-right: [w274] -> w257
              shift-left: w260 -> [w275]
              tunnel: w259 -> [w276]
              tunnel: T10 {"Description"="", "Attributes"=[], "Methods"=[]} -> [w272]
              shift-right: [w268] -> w242
              shift-left: T3[] [] -> [w270]
              n108 = Unbundle By Name(w269) -> ("Type"=w277:T4, "Name"=w273:string, "TypeSpecificData"=w271:variant)
              n109 = case shown="\"Class\", \"Interface\"" w277 {
                tunnel: w276 -> [_ w291]
                tunnel: w275 -> [w279 w290]
                tunnel: [w279 w288] -> w274
                tunnel: w273 -> [_ w287]
                tunnel: w272 -> [_ w286]
                tunnel: w271 -> [_ w285]
                tunnel: w270 -> [w278 w282]
                tunnel: w269 -> [_ w281]
                tunnel: [w278 w280] -> w268
                frame Default {
                }
                frame "Class", "Interface" {
                  n110 = Variant To Data(type=w286, Variant=w285) -> (data=w284:T10)  [unwired: 1 in, 1 out]
                  n111 = Unbundle By Name(w284) -> ("Description"=w283:string)
                  n112 = Bundle(cluster=w291, "Name"=w287, "Desc"=w283) -> (w289:cluster{"Name":string, "Desc":string})
                  n113 = Build Array (concatenate)(w282, w281) -> (w280:T3[])
                  n114 = Build Array (concatenate)(w290, w289) -> (w288:cluster{"Name":string, "Desc":string}[])
                }
              }
            }
            "Nodes" <- w257
            n115 = Empty Array?(array=w250) -> (empty?=w248:bool)
            n116 = Select(t=u8 0 ("Disabled"), s=w256, f=u8 2 ("Disabled")) -> (s? t:f=w255:u8)
            n117 = property on="Help" class="Bool"("Disabled"=w255) -> ()  [unwired: 2 in, 2 out]
            n118 = Select(t=u8 2 ("Disabled"), s=w248, f=u8 0 ("Disabled")) -> (s? t:f=w249:u8)
            n119 = property on="OK" class="Bool"("Disabled"=w249) -> ()  [unwired: 2 in, 2 out]
            n120 = Bundle By Name(cluster=w246, "ClassNodes"=w242) -> (w245:T6)
          }
          event "Refresh": Mouse Down {
            n121 = event-data() -> ("Mods.Double Click"=w292:bool)  [unwired: 1 out]
            n122 = case shown="True" w292 {
              frame False {
              }
              frame True {
                n123 = property on="Design Patterns" class="Tree (strict)"() -> (error out=w297:errorcluster, "Value"=w298:string)  [unwired: 2 in, 1 out]
                n124 = property on="Design Patterns" class="Tree (strict)"(error in=w297, "Val(Sgnl)"="" ("Value (Signaling)")) -> (error out=w296:errorcluster)  [unwired: 1 in, 1 out]
                n125 = property on="Design Patterns" class="Tree (strict)"(error in=w296, "Val(Sgnl)"=w298) -> ()  [unwired: 1 in, 2 out]
              }
            }
          }
          event "OpenPatternFile": Mouse Down {
            n126 = event-data() -> ("Mods.Double Click"=w303:bool)  [unwired: 1 out]
            n127 = case shown="True" w303 {
              tunnel: w302 -> [_ w311]
              tunnel: w301 -> [_ w309]
              frame False {
              }
              frame True {
                n128 = local read "NewVal"() -> (w310:string)
                n129 = Search 1D Array(1D array=w311, element=w310) -> (index of element=w312:i32)  [unwired: 1 out]
                n130 = Index Array(array=w309, index=w312) -> (element=w308:T16)
                n131 = Unbundle By Name(w308) -> ("PatternFile"=w307:path)
                n132 = Format Into String(format string="notepad \"%s\"", w307) -> (resulting string=w305:string)  [unwired: 2 in, 1 out]
                n133 = call <vilib>:"System Exec.vi"("wait until completion? (T)"=FALSE, "command line"=w305) -> ()  [unwired: 6 in, 4 out]
              }
            }
          }
          event "Help": Value Change {
            n134 = event-data() -> ()  [unwired: 7 out]
            n135 = local read "Design Patterns"() -> (w321:string)
            n136 = Search 1D Array(1D array=w322, element=w321) -> (index of element=w324:i32)  [unwired: 1 out]
            n137 = Index Array(array=w320, index=w324) -> (element=w323:T16)
            n138 = Unbundle By Name(w323) -> ("stripped path"=w313:path, "Pattern.Help"=w317:string)
            n139 = Match Pattern(string=w317, regular expression="http:") -> (offset past match=w318:i32)  [unwired: 4 out]
            n140 = case shown="-1" w318 {
              tunnel: w317 -> [w325 w328]
              tunnel: [w325 w326] -> w316
              tunnel: w313 -> [_ w329]
              frame 0, Default {
              }
              frame -1 {
                n141 = Build Path(base path=w329, name or relative path=w328) -> (appended path=w327:path)
                n142 = Path To String(path=w327) -> (string=w326:string)
              }
            }
            n143 = call-poly <vilib>:"Open URL in Default Browser.vi"("URL"=w316) -> ()  [unwired: 1 in, 6 out]
          }
          event Panel Close? {
            w330 = TRUE ("Discard?")
            n144 = event-data() -> ()  [unwired: 2 out]
            n145 = Bundle By Name(cluster=w332, "Cancelled"=w330) -> (w331:T6)
            n146 = event-data("Discard?"=w330) -> ()  [unwired: 1 in, 1 out]
          }
          event "Cancel", "OK": Value Change {
            n147 = event-data() -> ()  [unwired: 4 out]
            n148 = Unbundle By Name(w338) -> ("CtrlRefs"=w337:refnum<vi>[], "ClassNodes"=w336:T3[], "NodeIndexies"=w335:i32[])
            n149 = case shown="True" "OK" {
              tunnel: w337 -> [_ w347]
              tunnel: w336 -> [_ w346]
              tunnel: w335 -> [_ w345]
              tunnel: [_ w344] -> w334
              frame False {
              }
              frame True {
                n150 = for {
                  tunnel: w347 -> [w351] mode=indexing
                  tunnel: w346 -> [_] mode=indexing
                  tunnel: w345 -> [w350]
                  tunnel: [w348] -> w344 mode=indexing
                  n151 = property class="Ring (strict)"(reference=w351) -> ("Value"=w349:u16)  [unwired: 1 in, 2 out]
                  n152 = case shown="1.." w349 {
                    selector: w349 -> [_ w354]
                    tunnel: w350 -> [_ w356]
                    tunnel: [-1 w353] -> w348
                    frame 0, Default {
                    }
                    frame 1.. {
                      n153 = Decrement(x=w354) -> (x-1=w355:u16)
                      n154 = Index Array(array=w356, index=w355) -> (element=w353:i32)
                    }
                  }
                }
              }
            }
            n155 = Bundle By Name(cluster=w342, "Cancelled"="Cancel", "NodeIndexies"=w334) -> (w341:T6)
          }
        }
      }
      frame "Draw" {
        w362 = 1000
        w376 = 0.0 ("x")
        n156 = Unbundle By Name(w387) -> ("Graphics"=w371:refnum<class "Graphics.lvclass">, "Grid"=w373:refnum<class "Grid.lvclass">)
        n157 = Unbundle By Name(w387) -> ("PIDs"=w391:string[], "Patterns"=w390:T15)  [unwired: 1 out]
        n158 = local read "Design Patterns"() -> (w392:string)
        n159 = call <resource>:"ClassDiagramGraph_Create.vi"("error in (no error)"=w365) -> ("reference out"=w363:refnum<class "ClassDiagramGraph.lvclass">, "error out"=w364:errorcluster)  [unwired: 1 in, 16 out]
        n160 = Search 1D Array(1D array=w391, element=w392) -> (index of element=w394:i32)  [unwired: 1 out]
        n161 = Index Array(array=w390, index=w394) -> (element=w393:T16)
        n162 = Unbundle By Name(w393) -> ("Nodes"=w389:T3[], "Links"=w388:T1[])
        n163 = call <resource>:"DesignPatterns_DrawNodesAndLinks.vi"("GraphIn"=w363, "Graphics"=w371, "Grid"=w373, "Nodes"=w389, "Links"=w388, "error in (no error)"=w364, "Y-Offset"=w359, "X-Offset"=w360) -> ("GraphOut"=w386:refnum<class "ClassDiagramGraph.lvclass">, "error out"=w372:errorcluster)  [unwired: 9 in, 1 out]
        n164 = call-dynamic "layout.vi"("reference"=w386, "error in (no error)"=w372) -> ("reference out"=w377:refnum<class "ClassDiagramGraph.lvclass">, "error out"=w378:errorcluster)  [unwired: 16 in]
        n165 = call <resource>:"resetPicture.vi"("reference"=w371, "error in (no error)"=w378) -> ("reference out"=w384:refnum<class "Graphics.lvclass">, "error out"=w383:errorcluster)  [unwired: 16 out]
        n166 = call <resource>:"getScreenBounds.vi"("reference"=w384, "error in (no error)"=w383) -> ("reference out"=w361:refnum<class "Graphics.lvclass">, "bounds"=w381:T13, "ZoomChanged"=w380:bool, "error out"=w382:errorcluster)  [unwired: 14 out]
        n167 = Bundle(cluster=w381, "x"=w376, "y"=w376, "width"=w362, "height"=w362) -> (w375:T13)
        n168 = call-dynamic "draw.vi"("reference"=w373, "graphics"=w361, "bounds"=w375, "ForceRedrawGrid"=w380, "error in (no error)"=w382) -> ("reference out"=w374:refnum<class "Grid.lvclass">, "error out"=w385:errorcluster)  [unwired: 13 in]
        n169 = call-dynamic "draw.vi"("reference"=w377, "graphics"=w371, "grid"=w374, "error in (no error)"=w385, "SelectedNodes"=refnum<class "AbstractNode.lvclass">[] [], "HideOverLays(False)"=TRUE) -> ("reference out"=w366:refnum<class "ClassDiagramGraph.lvclass">, "error out"=w370:errorcluster)  [unwired: 10 in, 2 out]
        n170 = call <resource>:"updateScreen.vi"("reference"=w371, "error in (no error)"=w370) -> ("picture"=→"Picture":picture, "error out"=w368:errorcluster)  [unwired: 16 out]
        n171 = call-dynamic "Destroy.vi"("reference"=w366, "error in (no error)"=w368) -> ("error out"=w367:errorcluster)  [unwired: 17 in]
      }
      frame "PlaceControls" {
        n172 = Unbundle By Name(w399) -> ("CtrlRefs"=w400:refnum<vi>[], "ClassNodes"=w407:T3[])
        n173 = property on="Picture" class="Pict"() -> ("Left"=w413:i32, "Top"=w409:i32)  [unwired: 2 in, 2 out]
        n174 = Subtract(x=w411, y=25) -> (x-y=w408:i32)
        n175 = Add(x=w413, y=w412) -> (x+y=w398:i32)
        n176 = Add(x=w409, y=w408) -> (x+y=w406:i32)
        n177 = Add(x=w398, y=3) -> (x+y=w396:i32)
        n178 = for {
          tunnel: w400 -> [w434] mode=indexing
          tunnel: w407 -> [w433] mode=indexing
          tunnel: w396 -> [w430]
          tunnel: w406 -> [w427]
          shift-right: [w424] -> w402
          shift-left: w405 -> [w425]
          n179 = Unbundle By Name(w433) -> ("X"=w432:i32, "Y"=w429:i32)
          n180 = Add(x=w432, y=w430) -> (x+y=w431:i32)
          n181 = Add(x=w429, y=w427) -> (x+y=w428:i32)
          n182 = property class="Ring (strict)"(reference=w434, error in=w425, "Visible"=TRUE, "Left"=w431, "Top"=w428, "Value"=u16 0, "Disabled Items []"=i32[] []) -> (error out=w424:errorcluster)  [unwired: 1 out]
        }
        n183 = Empty Array?(array=w404) -> (empty?=w403:bool)
        n184 = Unbundle By Name(w399) -> ("ClassSelected"=w395:bool[])
        n185 = case shown="False" w403 {
          tunnel: w402 -> [w418 w422]
          tunnel: [w418 w422] -> w401
          tunnel: w400 -> [w419 _]
          tunnel: w395 -> [w417 _]
          frame False {
            n186 = Index Array(array=w419) -> ()  [unwired: 1 in, 1 out]
            n187 = Search 1D Array(1D array=w417, element=TRUE) -> (index of element=w415:i32)  [unwired: 1 in]
            n188 = case shown="0, Default" w415 {
              selector: w415 -> [w421 _]
              frame 0, Default {
                n189 = Increment(x=w421) -> (x+1=w420:i32)
                n190 = property on="Ring 1" class="Ring (strict)"("Val(Sgnl)"=w420) -> ()  [unwired: 2 in, 2 out]
              }
              frame -1 {
              }
            }
          }
          frame True {
          }
        }
      }
    }
    n191 = Equal?(x=w26, y="Exit") -> (x = y?=w29:bool)
    n192 = Select(t="Error", s=w25, f=w26) -> (s? t:f=w30:string)
  }
  "error out" <- w16
  n193 = stacked-sequence {
    tunnel: w6 -> [w436]
    tunnel: [w438] -> w4
    tunnel: [w437] -> w3
    tunnel: [w436] -> w2
    frame #0 {
      n194 = Unbundle By Name(w436) -> ("PIDs"=w442:string[], "Patterns"=w443:T15)
      n195 = local read "Design Patterns"() -> (w441:string)
      n196 = Search 1D Array(1D array=w442, element=w441) -> (index of element=w439:i32)  [unwired: 1 out]
      n197 = Index Array(array=w443, index=w439) -> (element=w440:T16)
      n198 = Unbundle By Name(w440) -> ("Nodes"=w438:T3[], "Links"=w437:T1[])
    }
  }
  "NodesOut" <- w4
  "LinksOut" <- w3
  n199 = Unbundle By Name(w2) -> ("NodeIndexies"=→"NodeIndexies":i32[])
  n200 = Unbundle By Name(w6) -> ("CtrlRefs"=w5:refnum<vi>[], "Cancelled"=→"Cancelled":bool, "Event"=w15:refnum<event-registration>)
  n201 = Unregister For Events(event registration refnum=w15) -> ()  [unwired: 1 in, 1 out]
  n202 = for {
    tunnel: w5 -> [w445] mode=indexing
    n203 = property class="Ring (strict)"(reference=w445, "Visible"=FALSE) -> ()  [unwired: 1 in, 2 out]
  }
  "GraphOut" <- "GraphIn"
